vi "FuncVI_Sub - Script - Link to Caller CSE instance.vi"(6 "Link(T)/Delink(F)":bool, 7 "Caller CSE RefNum":T2, 8 "error in":errorcluster, 10 "Callback VI RefNum":T1, 11 "CSE RefNum":T2) -> (0 "error out":errorcluster, 2 "Callback VI RefNum out":T1, 3 "dup CSE RefNum":T2)   [LabVIEW 2021]
doc: "::: CalcExpress Toolkit :::\nCopyright (c) 2000-2026 Konstantin Shifershteyn. All rights reserved."
uses:
  cse.llb/CSE Instance RefNum.ctl
  cse.llb/CSE Callback VI RefNum.ctl
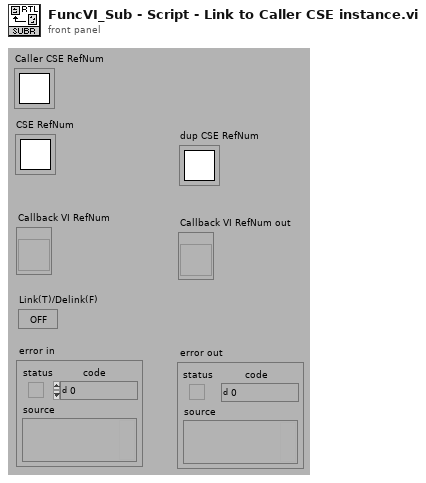
[diagram p1: front panel]
types:
  T1 = typedef "CSE Callback VI RefNum.ctl" = refnum<vi>
  T2 = typedef "CSE Instance RefNum.ctl" = refnum<k1>
  T3 = typedef "CSE Type - Run Mode.ctl" = u32
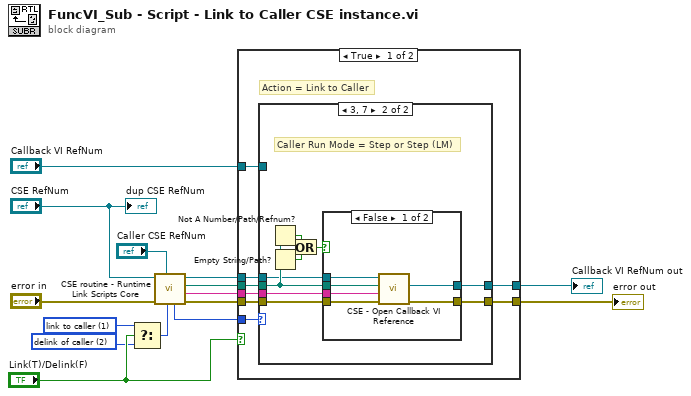
[diagram p0: block diagram]
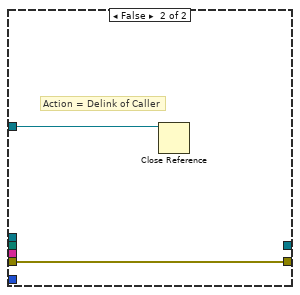
[diagram p4: hidden frame]
diagram:
  w1 = 2 items=["save vi path", "link to caller", "delink of caller", "call-chain info"] ("action")
  w2 = 1 items=["save vi path", "link to caller", "delink of caller", "call-chain info"] ("action")
  n1 = Select(t=w2, s="Link(T)/Delink(F)", f=w1) -> (s? t:f=w4:i32)
  n2 = call "CSE routine - Runtime Link Scripts Core.vi"("action"=w4, "Caller CSE RefNum"="Caller CSE RefNum", "error in"="error in", "CSE RefNum"="CSE RefNum") -> ("error out"=w12:errorcluster, "Script Name"=w6:string, "Callback VI Path out"=w7:path, "dup CSE RefNum"=w5:T2, "Caller Run mode"=w8:T3)  [unwired: 2 in, 1 out]
  n3 = case shown="True" "Link(T)/Delink(F)" {
    tunnel: w12 -> [w23 w43]
    tunnel: [w22 w43] -> w15
    tunnel: w7 -> [w21 _]
    tunnel: "Callback VI RefNum" -> [w20 w42]
    tunnel: [w19 _] -> w13
    tunnel: w8 -> [w18 _]
    tunnel: w6 -> [w17 _]
    tunnel: w5 -> [w16 _]
    frame True {
      # "Action = Link to Caller"
      n4 = case shown="3, 7" w18 {
        tunnel: w23 -> [w25 w31]
        tunnel: [w25 w30] -> w22
        tunnel: w21 -> [_ w29]
        tunnel: w20 -> [w24 _]
        tunnel: [w24 w28] -> w19
        tunnel: w17 -> [_ w27]
        tunnel: w16 -> [_ w26]
        frame 0, Default {
        }
        frame 3, 7 {
          # "Caller Run Mode = Step or Step (LM)"
          n5 = Not A Number/Path/Refnum?(number/path/refnum=w29) -> (NaN/Path/Refnum?=w34:bool)
          n6 = Empty String/Path?(string/path=w29) -> (empty?=w33:bool)
          n7 = Or(x=w34, y=w33) -> (x .or. y?=w32:bool)
          n8 = case shown="False" w32 {
            tunnel: w31 -> [w40 w41]
            tunnel: [w37 w41] -> w30
            tunnel: w29 -> [w38 _]
            tunnel: [w35 _] -> w28
            tunnel: w27 -> [w39 _]
            tunnel: w26 -> [w36 _]
            frame False {
              n9 = call "CSE - Open Callback VI Reference.vi"("error in"=w40, "Window Title"=w39, "Callback VI Path"=w38, "CSE RefNum"=w36) -> ("error out"=w37:errorcluster, "Callback VI RefNum"=w35:T1)  [unwired: 5 in, 1 out]
            }
            frame True {
            }
          }
        }
      }
    }
    frame False {
      # "Action = Delink of Caller"
      n10 = Close Reference(reference=w42) -> ()  [unwired: 1 in, 1 out]
    }
  }
  "error out" <- w15
  "Callback VI RefNum out" <- w13
  "dup CSE RefNum" <- "CSE RefNum"
